vi "DI Pulse Check.vi"(8 "Min Pulse Off Time [CAD]":sgl, 9 "Engine Speed [RPM]":sgl, 11 "DI Cluster":T1) -> (0 "DI Pulse Overlap Error":bool)   [LabVIEW 2015, in "ECS-RT.lvlib"]
uses:
  ECS-RT.lvlib
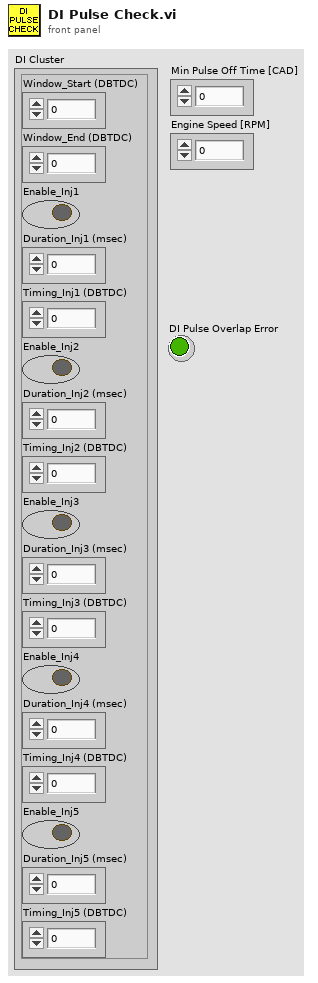
[diagram p1: front panel]
types:
  T1 = cluster{"Window_Start (DBTDC)":sgl, "Window_End (DBTDC)":sgl, "Enable_Inj1":bool, "Duration_Inj1 (msec)":sgl, "Timing_Inj1 (DBTDC)":sgl, "Enable_Inj2":bool, "Duration_Inj2 (msec)":sgl, "Timing_Inj2 (DBTDC)":sgl, "Enable_Inj3":bool, "Duration_Inj3 (msec)":sgl, "Timing_Inj3 (DBTDC)":sgl, "Enable_Inj4":bool, "Duration_Inj4 (msec)":sgl, "Timing_Inj4 (DBTDC)":sgl, "Enable_Inj5":bool, "Duration_Inj5 (msec)":sgl, "Timing_Inj5 (DBTDC)":sgl}
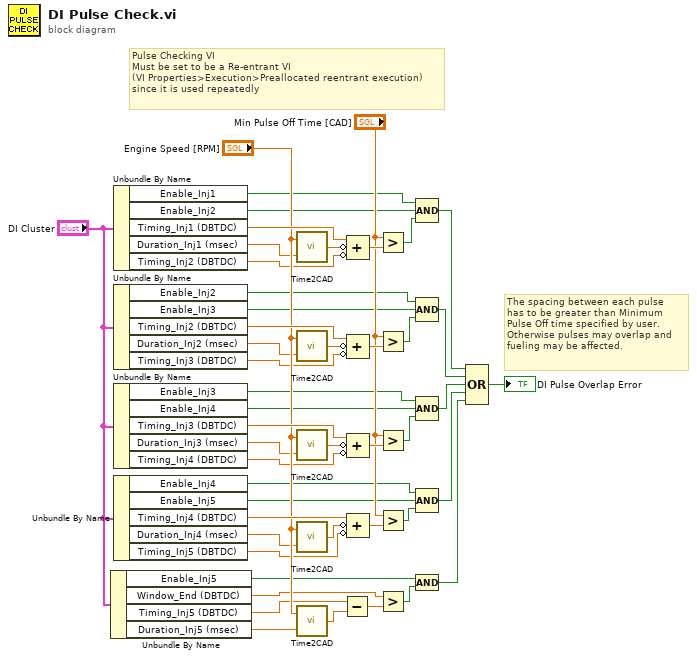
[diagram p0: block diagram]
diagram:
  # "Pulse Checking VI\nMust be set to be a Re-entrant VI \n(VI Properties>Execution>Preallocated reentrant execution)\nsince it is used repeatedly"
  # "The spacing between each pulse\nhas to be greater than Minimum \nPulse Off time specified by user.\nOtherwise pulses may overlap and\nfueling may be affected."
  n1 = Unbundle By Name("DI Cluster") -> ("Enable_Inj5"=w3:bool, "Window_End (DBTDC)"=w20:sgl, "Timing_Inj5 (DBTDC)"=w33:sgl, "Duration_Inj5 (msec)"=w21:sgl)
  n2 = Unbundle By Name("DI Cluster") -> ("Enable_Inj1"=w10:bool, "Enable_Inj2"=w11:bool, "Timing_Inj1 (DBTDC)"=w48:sgl, "Duration_Inj1 (msec)"=w29:sgl, "Timing_Inj2 (DBTDC)"=w28:sgl)
  n3 = Unbundle By Name("DI Cluster") -> ("Enable_Inj2"=w14:bool, "Enable_Inj3"=w15:bool, "Timing_Inj2 (DBTDC)"=w43:sgl, "Duration_Inj2 (msec)"=w27:sgl, "Timing_Inj3 (DBTDC)"=w26:sgl)
  n4 = Unbundle By Name("DI Cluster") -> ("Enable_Inj3"=w19:bool, "Enable_Inj4"=w18:bool, "Timing_Inj3 (DBTDC)"=w37:sgl, "Duration_Inj3 (msec)"=w25:sgl, "Timing_Inj4 (DBTDC)"=w24:sgl)
  n5 = Unbundle By Name("DI Cluster") -> ("Enable_Inj4"=w6:bool, "Enable_Inj5"=w7:bool, "Timing_Inj4 (DBTDC)"=w38:sgl, "Duration_Inj4 (msec)"=w23:sgl, "Timing_Inj5 (DBTDC)"=w22:sgl)
  n6 = call <vilib>:"Time2CAD.vi"("Time [ms]"=w29, "Speed (RPM)"="Engine Speed [RPM]") -> ("CAD"=w47:sgl)
  n7 = call <vilib>:"Time2CAD.vi"("Time [ms]"=w27, "Speed (RPM)"="Engine Speed [RPM]") -> ("CAD"=w44:sgl)
  n8 = call <vilib>:"Time2CAD.vi"("Time [ms]"=w25, "Speed (RPM)"="Engine Speed [RPM]") -> ("CAD"=w42:sgl)
  n9 = call <vilib>:"Time2CAD.vi"("Time [ms]"=w23, "Speed (RPM)"="Engine Speed [RPM]") -> ("CAD"=w39:sgl)
  n10 = call <vilib>:"Time2CAD.vi"("Time [ms]"=w21, "Speed (RPM)"="Engine Speed [RPM]") -> ("CAD"=w34:sgl)
  n11 = Subtract(x=w33, y=w34) -> (x-y=w32:sgl)
  n12 = Compound Arithmetic op=ADD(w48, invert w47, invert w28) -> (w46:sgl)
  n13 = Compound Arithmetic op=ADD(w43, invert w44, invert w26) -> (w45:sgl)
  n14 = Compound Arithmetic op=ADD(w37, invert w42, invert w24) -> (w41:sgl)
  n15 = Compound Arithmetic op=ADD(w38, invert w39, invert w22) -> (w40:sgl)
  n16 = Greater?(x="Min Pulse Off Time [CAD]", y=w46) -> (0:w9:bool)
  n17 = Greater?(x="Min Pulse Off Time [CAD]", y=w45) -> (0:w13:bool)
  n18 = Greater?(x="Min Pulse Off Time [CAD]", y=w41) -> (0:w17:bool)
  n19 = Greater?(x="Min Pulse Off Time [CAD]", y=w40) -> (0:w5:bool)
  n20 = Greater?(x=w20, y=w32) -> (0:w2:bool)
  n21 = Compound Arithmetic op=AND(w10, w11, w9) -> (w8:bool)
  n22 = Compound Arithmetic op=AND(w14, w15, w13) -> (w12:bool)
  n23 = Compound Arithmetic op=AND(w19, w18, w17) -> (w16:bool)
  n24 = Compound Arithmetic op=AND(w6, w7, w5) -> (w4:bool)
  n25 = Compound Arithmetic op=AND(w3, w2) -> (w1:bool)
  n26 = Compound Arithmetic op=OR(w8, w12, w16, w4, w1) -> (→"DI Pulse Overlap Error":bool)
